vi "VIH Constant - HHP Template File.vi"() -> (3 "HHP Template File path":path)   [LabVIEW 2014]
doc: "::: VI Helpeks :::\nCopyright (c) 2000-2026 Konstantin Shifershteyn. All rights reserved."
panel:
  # "VI Helpeks\nCopyright (c) 2012-2026 Konstantin Shifershteyn"
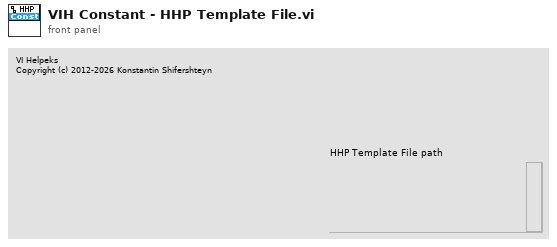
[diagram p1: front panel]
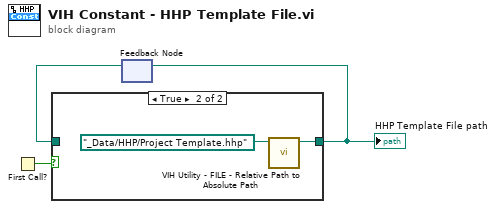
[diagram p0: block diagram]
diagram:
  n1 = First Call?() -> (First Call?: T/F=w3:bool)
  n2 = feedback #1() -> (w2:path)  [unwired: 1 in]
  n3 = case shown="True" w3 {
    tunnel: [w4 w5] -> w1
    tunnel: w2 -> [w4 _]
    frame False {
    }
    frame True {
      n4 = call "VIH Utility - FILE - Relative Path to Absolute Path.vi"("Path"=path "_Data/HHP/Project Template.hhp" ("Template HHP File")) -> ("Path out"=w5:path)  [unwired: 9 in, 1 out]
    }
  }
  "HHP Template File path" <- w1
  n5 = feedback-in #1(w1) -> ()
